vi "Index Project Item by Name.vi"(8 "error in":errorcluster, 10 "Name":string, 11 "Project Items":refnum<vi>[](array[refnum])) -> (0 "error out":errorcluster, 3 "Project Item":refnum<vi>)   [LabVIEW 2026]
doc: "Extract reference of project item specified by name. If the item is not found this VI produces an error."
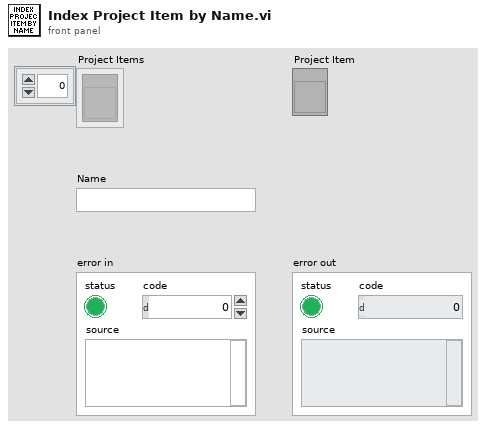
[diagram p1: front panel]
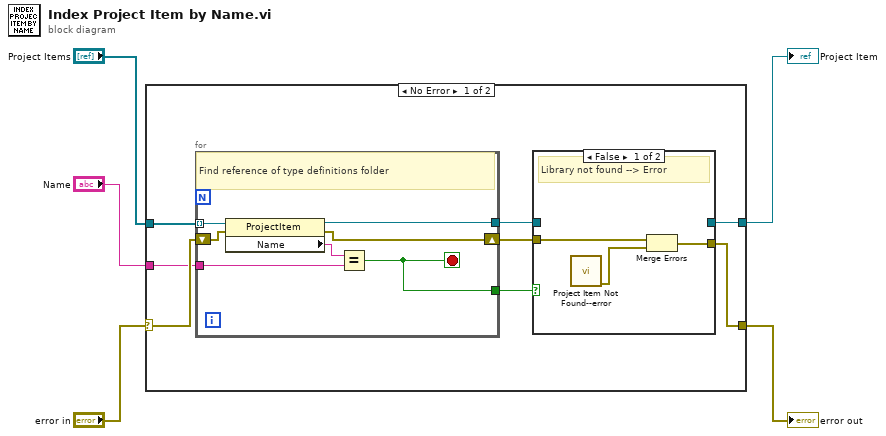
[diagram p0: block diagram]
diagram:
  n1 = case shown="No Error" "error in" {
    selector: "error in" -> [w11 w26]
    tunnel: "Project Items" -> [w9 _]
    tunnel: [w12 w26] -> w5
    tunnel: "Name" -> [w7 _]
    tunnel: [w6 _] -> w1
    frame No Error {
      n2 = for {
        tunnel: w9 -> [w23] mode=indexing
        tunnel: w7 -> [w21]
        shift-right: [w24] -> w13
        shift-left: w11 -> [w25]
        tunnel: [w20] -> w8
        tunnel: [w19] -> w10
        stop <- w19 stop-if-true
        # "Find reference of type definitions folder"
        n3 = property class="ProjectItem"(reference=w23, error in=w25) -> (reference out=w20:refnum<vi>, error out=w24:errorcluster, "Name"=w22:string)
        n4 = Equal?(x=w22, y=w21) -> (x = y?=w19:bool)
      }
      n5 = case shown="False" w10 {
        tunnel: w13 -> [w16 w18]
        tunnel: w8 -> [_ w17]
        tunnel: [_ w17] -> w6
        tunnel: [w14 w18] -> w12
        frame False {
          # "Library not found --> Error"
          n6 = call "Project Item Not Found--error.vi"() -> ("error out"=w15:errorcluster)  [unwired: 11 in]
          n7 = Merge Errors(w16, w15) -> (w14:errorcluster)
        }
        frame True {
          # "Library found"
        }
      }
    }
    frame Error {
      # "Pass error without further action."
    }
  }
  "error out" <- w5
  "Project Item" <- w1
